vi "RemoteVI Menu Hover.vi"(0 "hWnd":u64, 5 "popup open?":bool, 7 "clicked?":bool) -> ()   [LabVIEW 2020, in "RemoteVI.lvlib"]
doc: "The hover part of one server loop iteration (docs\\architecture.md, Popups): makes the remote pointer act on open LabVIEW menus as a local pointer does, without moving the host cursor or any window. The pointer position comes from RemoteVI Menu Pointer.vi (RemoteVI Note Popup Pointer.vi stores each WM_MOUSEMOVE a client sends while a popup is open, so a burst of moves is coalesced to the latest one). While a popup is open and a position waits, RemoteVI Hover Menus.vi does one step with keys: over the DEEPEST menu the highlight is moved onto the item under the pointer (VK_DOWN / VK_UP), and when it has stayed on one item for 400 ms VK_RIGHT is posted once - it opens that item's submenu next to its parent as a local hover does, and does nothing on an item without one (measured); over a PARENT of open submenus nothing happens on the item that opened the submenu, elsewhere after 300 ms of rest the submenus are closed with VK_LEFT and the parent's highlight follows. A popup that takes no keys (colour picker, line width popup) gets no hover. In an iteration in which a client clicked (clicked?) no step is made - the click has just set the state. When no popup is open the state is reset, except swallow up (the button-up of a click that chose a menu item). Win32 only, no VI Server call; errors are dropped."
uses:
  RemoteVI.lvlib
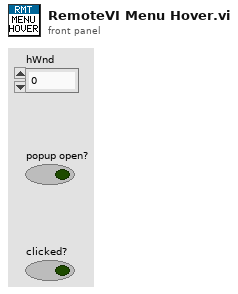
[diagram p1: front panel]
types:
  T1 = cluster{"active":bool, "x":i32, "y":i32, "moved":u32, "navigated":bool, "menu":u64, "top":i32, "hit":bool, "row since":u32, "dwelled":bool, "plain":u64, "swallow up":bool}
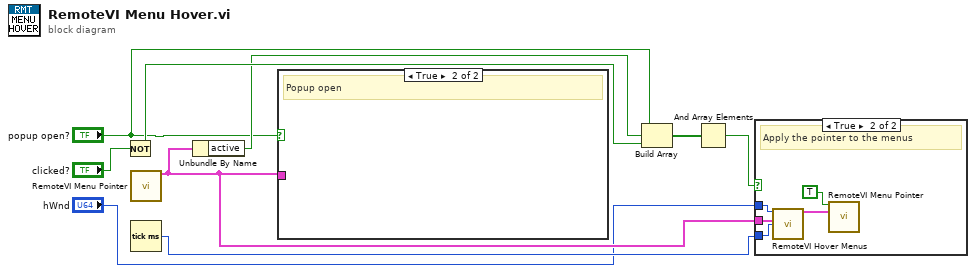
[diagram p0: block diagram]
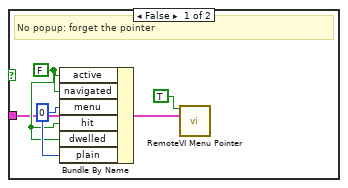
[diagram p3: hidden frame]
diagram:
  n1 = Not(x="clicked?") -> (.not. x?=w7:bool)
  n2 = call "RemoteVI Menu Pointer.vi"() -> ("state"=w5:T1)  [unwired: 15 in]
  n3 = Tick Count (ms)() -> (millisecond timer value=w4:u32)
  n4 = Unbundle By Name(w5) -> ("active"=w6:bool)
  n5 = case shown="True" "popup open?" {
    tunnel: w5 -> [w10 _]
    frame False {
      w13 = u64 0
      w11 = FALSE
      # "No popup: forget the pointer"
      n6 = Bundle By Name(cluster=w10, "active"=w11, "navigated"=w11, "menu"=w13, "hit"=w11, "dwelled"=w11, "plain"=w13) -> (w14:T1)
      n7 = call "RemoteVI Menu Pointer.vi"("write?"=TRUE, "state in"=w14) -> ()  [unwired: 13 in, 1 out]
    }
    frame True {
      # "Popup open"
    }
  }
  n8 = Build Array("popup open?", w6, w7) -> (w8:bool[])
  n9 = And Array Elements(Boolean array=w8) -> (logical AND=w9:bool)
  n10 = case shown="True" w9 {
    tunnel: "hWnd" -> [_ w16]
    tunnel: w5 -> [_ w15]
    tunnel: w4 -> [_ w17]
    frame False {
    }
    frame True {
      # "Apply the pointer to the menus"
      n11 = call "RemoteVI Hover Menus.vi"("hWnd"=w16, "state"=w15, "now"=w17) -> ("state out"=w18:T1)  [unwired: 12 in]
      n12 = call "RemoteVI Menu Pointer.vi"("write?"=TRUE, "state in"=w18) -> ()  [unwired: 13 in, 1 out]
    }
  }
